vi "1. Used as parameters parsed by CSM.vi"() -> ()   [LabVIEW 2017]
doc: "### Overview\n\nCSM INI Variable Support provides CSM with simple and easy-to-use configuration file support, enabling users to configure applications without explicitly reading or writing configuration files.\n\nThis example demonstrates how to use the INI Variable Support parsable parameters feature within CSM.\n\n### Introduction\n\nThis example shows how to use the CSM INI Variable Support feature to store parameter information in an INI configuration file. INI variables use the CSM API String format.\n\nVariable Syntax: `${section.variable:defaultValue}`\n\n- **section:** The section name in the configuration file. The `section` parameter is optional. If omitted, the default configuration section `SectionName=LabVIEW` is used.\n- **variable:** The variable name in the configuration file.\n- **defaultValue:** The default value used when the variable is not defined in the configuration file. The `defaultValue` is optional. If unspecified, it defaults to an empty string (`\"\"`).\n\n### Steps\n\n- Step1: Generate a temporary INI file and load it using the CSM - Load Configuration Variables From File VI.\n\n- Step2: Simulate a CSM module using a regular loop and use the CSM - Populate Configuration Variables VI to parse variables within a string into actual values. After running, compare the information displayed on the front panel with the comments to verify consistency.\n\n - Step2.1: In the code for this part, note that the section/variable does not exist in the configuration information.\n - Step2.2: Expected result for the code execution in Step2.1.\n - Step2.3: In the code for this part, note that CSM INI Variable Support is not limited to parameters. It can be used with any field.\n - Step2.4: Expected result for the code execution in Step2.3."
uses:
  INI-Static-Variable-Support/INI-Static-Variable-Support.lvlib
panel:
  out "State Queue":string
  # "#CSM-Example overview\n\nCSM INI Variable Support provides CSM with simple and easy-to-use configuration file support, enabling users to configure applications without explicitly reading or writing configuration files.\n\nThis example demonstrates how to use the INI Variable Support parsable parameters feature within CSM."
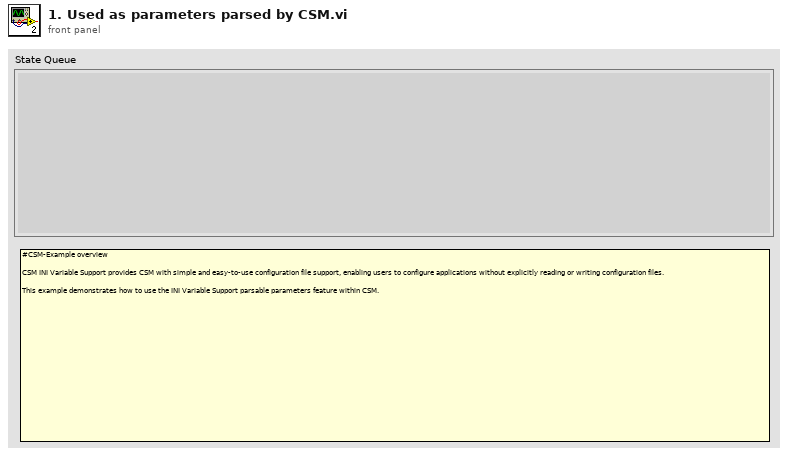
[diagram p1: front panel]
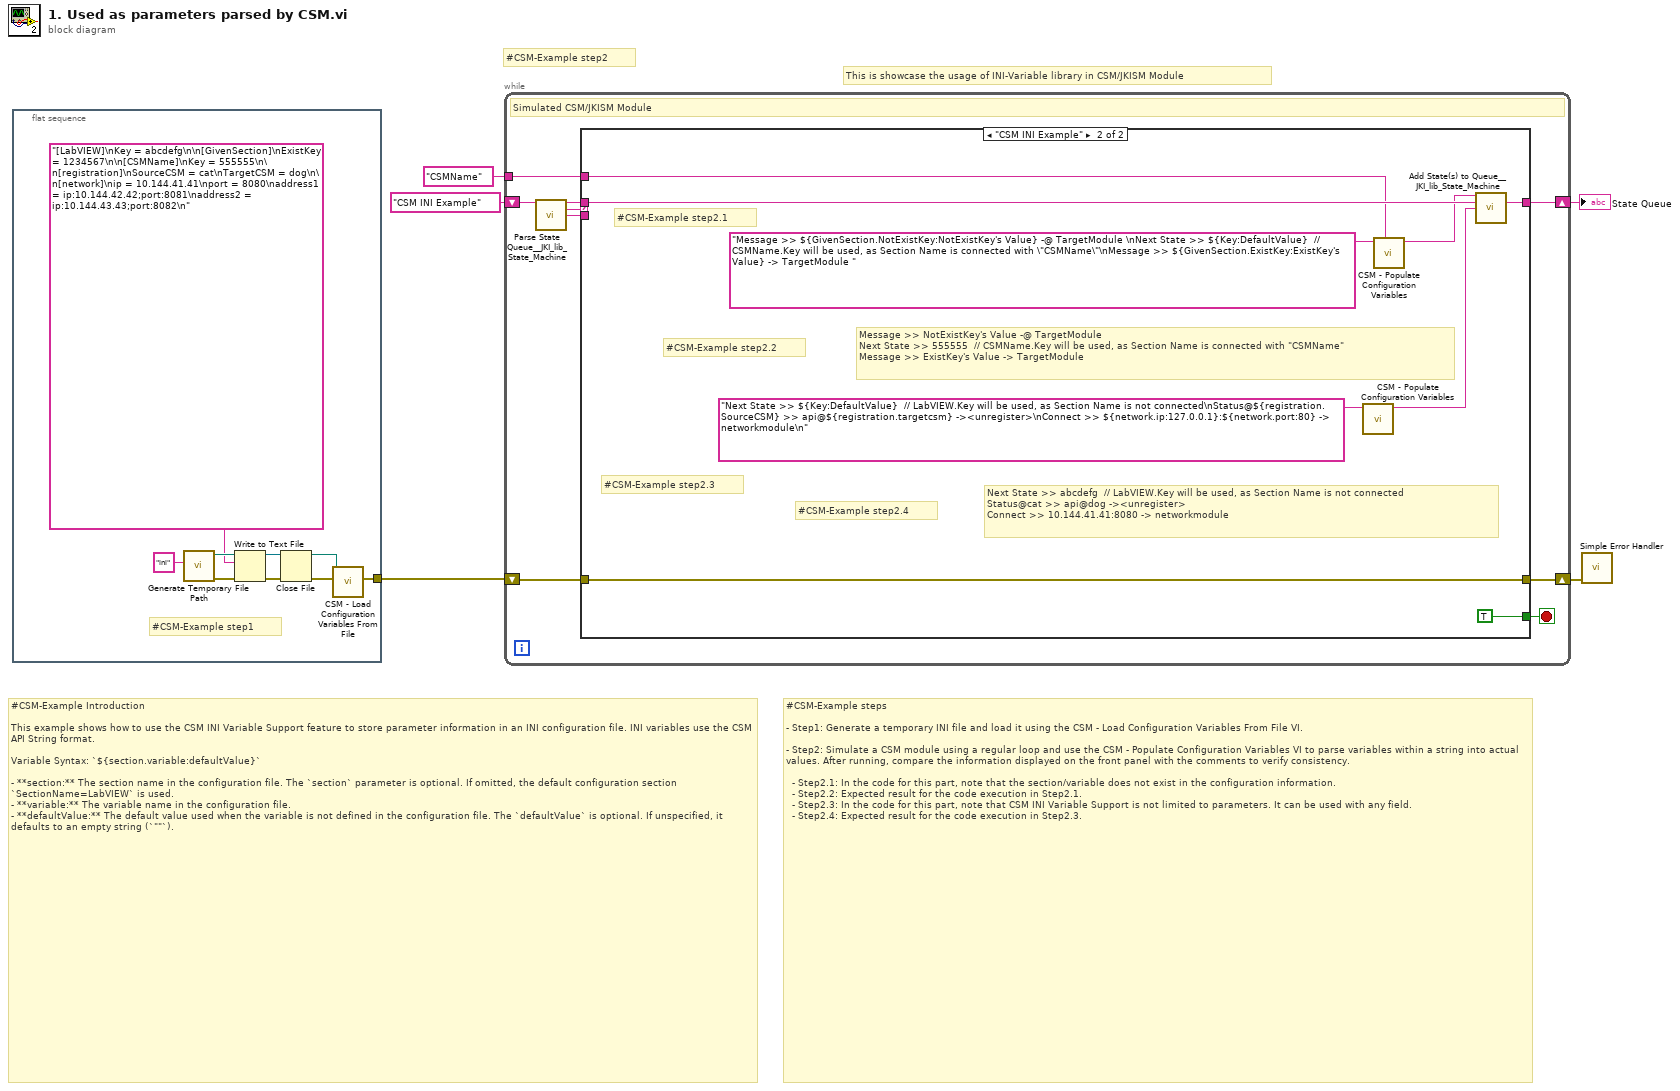
[diagram p0: block diagram]
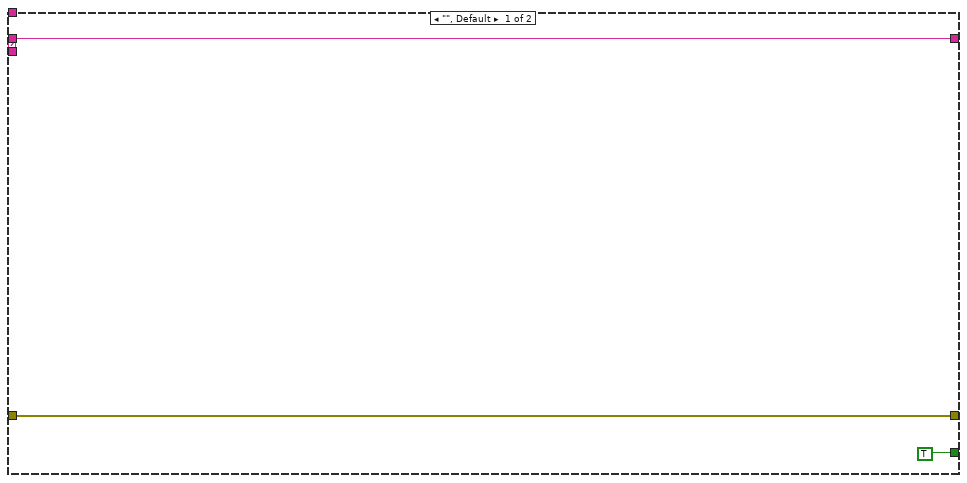
[diagram p2: hidden frame]
diagram:
  # "#CSM-Example step2"
  # "#CSM-Example steps\n\n- Step1: Generate a temporary INI file and load it using the CSM - Load Configuration Variables From File VI.\n\n- Step2: Simulate a CSM module using a regular loop and use the CSM - Populate Configuration Variables VI to parse variables within a string into actual values. After running, compare the information displayed on the front panel with the comments to verify consistency.\n\n  - Step2.1: In the code for this part, note that the section/variable does not exist in the configuration information.\n  - Step2.2: Expected result for the code execution in Step2.1.\n  - Step2.3: In the code for this part, note that CSM INI Variable Support is not limited to parameters. It can be used with any field.\n  - Step2.4: Expected result for the code execution in Step2.3."
  # "#CSM-Example Introduction\n\nThis example shows how to use the CSM INI Variable Support feature to store parameter information in an INI configuration file. INI variables use the CSM API String format.\n\nVariable Syntax: `${section.variable:defaultValue}`\n\n- **section:** The section name in the configuration file. The `section` parameter is optional. If omitted, the default configuration section `SectionName=LabVIEW` is used.\n- **variable:** The variable name in the configuration file.\n- **defaultValue:** The default value used when the variable is not defined in the configuration file. The `defaultValue` is optional. If unspecified, it defaults to an empty string (`\"\"`)."
  # "This is showcase the usage of INI-Variable library in CSM/JKISM Module"
  n1 = flat-sequence {
    tunnel: [w8] -> w2
    frame #0 {
      # "#CSM-Example step1"
      n2 = call <vilib>:"Generate Temporary File Path.vi"("Temporary File Extension (tmp)"="ini") -> ("error out"=w14:errorcluster, "Unique Temporary File Path"=w11:path)  [unwired: 9 in]
      n3 = Write to Text File(file (use dialog)=w11, text="[LabVIEW]\nKey = abcdefg\n\n[GivenSection]\nExistKey = 1234567\n\n[CSMName]\nKey = 555555\n\n[registration]\nSourceCSM = cat\nTargetCSM = dog\n\n[network]\nip = 10.144.41.41\nport = 8080\naddress1 = ip:10.144.42.42;port:8081\naddress2 = ip:10.144.43.43;port:8082\n", error in=w14) -> (refnum out=w10:refnum<file>, error out=w12:errorcluster)  [unwired: 1 in, 1 out]
      n4 = Close File(refnum=w10, error in=w12) -> (path=w6:path, error out=w9:errorcluster)
      n5 = call "CSM - Load Configuration Variables From File.vi"("error in (no error)"=w9, "Configuration Path"=w6) -> ("error out"=w8:errorcluster)  [unwired: 7 in]
    }
  }
  n6 = while "Communicable State Machine(CSM) 2025" {
    shift-right: [w21] -> w4
    shift-left: "CSM INI Example" ("State Queue") -> [w23]
    shift-right: [w16] -> w1
    shift-left: w2 -> [w17]
    tunnel: "CSMName" ("State Queue") -> [w15]
    stop <- w18 stop-if-true
    # "Simulated CSM/JKISM Module"
    n7 = call <vilib>:"Parse State Queue__JKI_lib_State_Machine.vi"("State Queue"=w23) -> ("Remaining States"=w22:string, "Current State"=w20:string, "Arguments"=w19:string)  [unwired: 12 in]
    n8 = case shown="\"CSM INI Example\"" w20 {
      tunnel: w22 -> [w26 w33]
      tunnel: [w26 w32] -> w21
      tunnel: w19 -> [_ _]
      tunnel: [TRUE TRUE] -> w18
      tunnel: w17 -> [w24 w34]
      tunnel: [w24 w34] -> w16
      tunnel: w15 -> [_ w29]
      frame "", Default {
      }
      frame "CSM INI Example" {
        # "#CSM-Example step2.4"
        # "#CSM-Example step2.3"
        # "#CSM-Example step2.2"
        # "#CSM-Example step2.1"
        # "Message >> NotExistKey's Value -@ TargetModule \nNext State >> 555555  // CSMName.Key will be used, as Section Name is connected with \"CSMName\"\nMessage >> ExistKey's Value -> TargetModule"
        # "Next State >> abcdefg  // LabVIEW.Key will be used, as Section Name is not connected\nStatus@cat >> api@dog -><unregister>\nConnect >> 10.144.41.41:8080 -> networkmodule"
        n9 = call "CSM - Populate Configuration Variables.vi"("String with INI-Variable"="Next State >> ${Key:DefaultValue}  // LabVIEW.Key will be used, as Section Name is not connected\nStatus@${registration.SourceCSM} >> api@${registration.targetcsm} -><unregister>\nConnect >> ${network.ip:127.0.0.1}:${network.port:80} -> networkmodule\n" ("String in")) -> ("String"=w27:string)  [unwired: 7 in, 1 out]
        n10 = call "CSM - Populate Configuration Variables.vi"("Section Name (\"\" as Default)"=w29, "String with INI-Variable"="Message >> ${GivenSection.NotExistKey:NotExistKey's Value} -@ TargetModule \nNext State >> ${Key:DefaultValue}  // CSMName.Key will be used, as Section Name is connected with \"CSMName\"\nMessage >> ${GivenSection.ExistKey:ExistKey's Value} -> TargetModule " ("String in")) -> ("String"=w31:string)  [unwired: 6 in, 1 out]
        n11 = call <vilib>:"Add State(s) to Queue__JKI_lib_State_Machine.vi"("State(s) in Front (\"\")"=w31, "State(s) in (\"\")"=w33, "State(s) at Back (\"\")"=w27) -> ("States Out"=w32:string)  [unwired: 12 in]
      }
    }
  }
  "State Queue" <- w4
  n12 = call <vilib>:"Simple Error Handler.vi"("error in (no error)"=w1) -> ()  [unwired: 4 in, 5 out]
